vi "Delete User from All Groups.vi"(5 "Save File":bool=TRUE, 6 "error in (no error)":errorcluster, 8 "LoginName":string, 9 "EasyUserManager in":refnum<class "EasyUserManager.lvclass">) -> (0 "error out":errorcluster, 3 "EasyUserManager out":refnum<class "EasyUserManager.lvclass">)   [LabVIEW 2024, in "EasyUserManager.lvclass"]
doc: "Remove the user specified by <B>LoginName</B> from all groups of which it is a member. \n\nThe boolean input <B>Save File</B> controls whether changes are immediately saved to the users file (Default: True)."
uses:
  EasyUserManager.lvclass
  EasyUserManager.lvclass/EasyUserManager.ctl
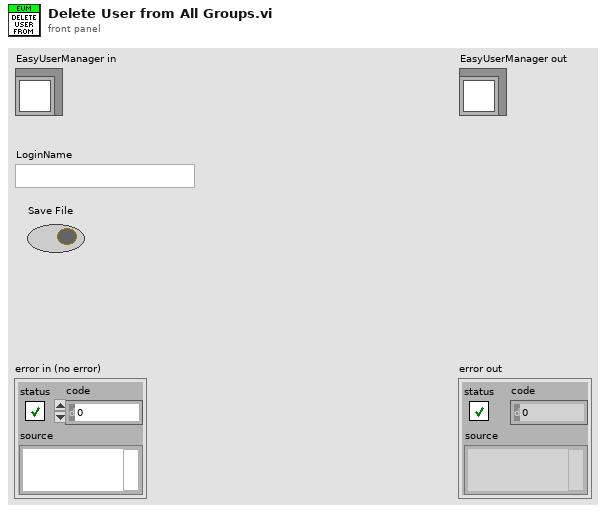
[diagram p1: front panel]
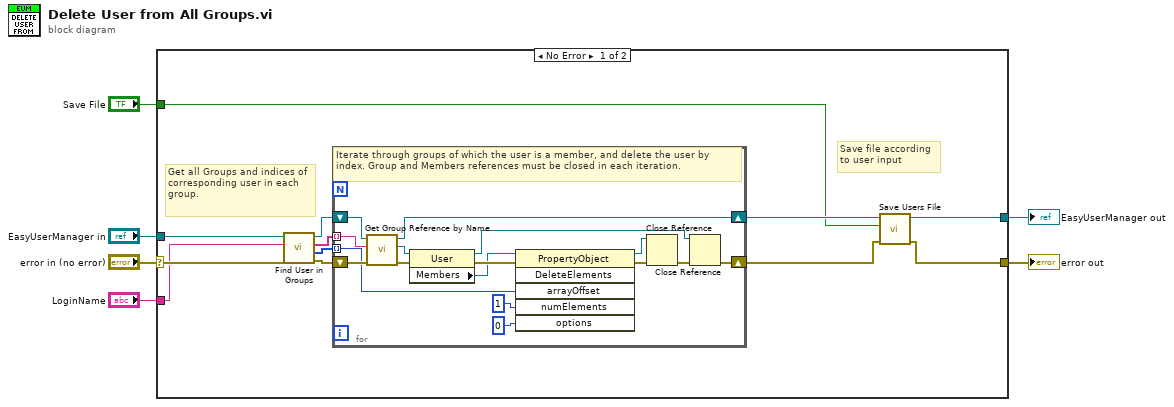
[diagram p0: block diagram]
diagram:
  n1 = case shown="No Error" "error in (no error)" {
    selector: "error in (no error)" -> [w9 w36]
    tunnel: [w10 w36] -> w5
    tunnel: [w12 w35] -> w3
    tunnel: "EasyUserManager in" -> [w18 w35]
    tunnel: "LoginName" -> [w8 _]
    tunnel: "Save File" -> [w7 _]
    frame No Error {
      # "Save file according\nto user input"
      # "Get all Groups and indices of corresponding user in each group."
      n2 = call "Find User in Groups.vi"("error in (no error)"=w9, "LoginName"=w8, "EasyUserManager in"=w18) -> ("error out"=w17:errorcluster, "Indexes"=w15:i32[], "Groups"=w16:string[], "EasyUserManager out"=w14:refnum<class "EasyUserManager.lvclass">)  [unwired: 1 in]
      n3 = for {
        shift-right: [w30] -> w11
        shift-left: w17 -> [w32]
        tunnel: w16 -> [w31] mode=indexing
        tunnel: w15 -> [w29] mode=indexing
        shift-right: [w33] -> w13
        shift-left: w14 -> [w34]
        # "Iterate through groups of which the user is a member, and delete the user by index. Group and Members references must be closed in each iteration."
        n4 = call "Get Group Reference by Name.vi"("error in (no error)"=w32, "Group Name"=w31, "EasyUserManager in"=w34) -> ("error out"=w20:errorcluster, "Group Reference"=w19:refnum<k7>, "EasyUserManager out"=w33:refnum<class "EasyUserManager.lvclass">)  [unwired: 2 in]
        n5 = property on="Property Node" class="User"(reference=w19, error in=w20) -> (reference out=w27:refnum<k7>, error out=w24:errorcluster, "Members"=w23:refnum<k7>)
        n6 = invoke on="Invoke Node" class="PropertyObject" method="DeleteElements"(reference=w23, error in=w24, "arrayOffset"=w29, "numElements"=1, "options"=0) -> (reference out=w25:refnum<k7>, error out=w26:errorcluster)  [unwired: 1 in, 4 out]
        n7 = Close Reference(reference=w25, error in (no error)=w26) -> (error out=w28:errorcluster)
        n8 = Close Reference(reference=w27, error in (no error)=w28) -> (error out=w30:errorcluster)
      }
      n9 = call "Save Users File.vi"("error in (no error)"=w11, "Save"=w7, "EasyUserManager in"=w13) -> ("error out"=w10:errorcluster, "EasyUserManager out"=w12:refnum<class "EasyUserManager.lvclass">)  [unwired: 3 in]
    }
    frame Error {
      # "Pass error and do nothing."
    }
  }
  "error out" <- w5
  "EasyUserManager out" <- w3
